vi "RGB to Colour.vi"(8 "error in (no error)":errorcluster, 9 "Blue":u8, 10 "Green":u8, 11 "Red":u8) -> (0 "error out":errorcluster, 3 "Color":u32(colorbox))   [LabVIEW 2018, in "Colour Lab.lvlib"]
uses:
  Colour Lab.lvlib
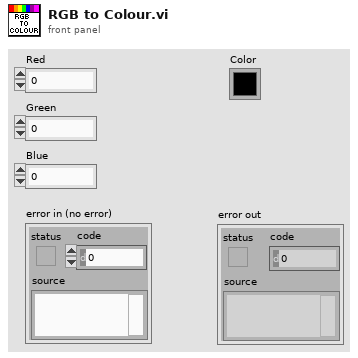
[diagram p1: front panel]
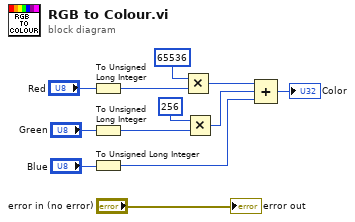
[diagram p0: block diagram]
diagram:
  n1 = To Unsigned Long Integer(number="Red") -> (unsigned 32bit integer=w8:u32)
  n2 = To Unsigned Long Integer(number="Green") -> (unsigned 32bit integer=w6:u32)
  n3 = To Unsigned Long Integer(number="Blue") -> (unsigned 32bit integer=w4:u32)
  n4 = Multiply(x=u32 65536 ("x^2"), y=w8) -> (x*y=w7:u32)
  n5 = Multiply(x=u32 256, y=w6) -> (x*y=w5:u32)
  n6 = Compound Arithmetic op=ADD(w7, w5, w4) -> (→"Color":u32)
  "error out" <- "error in (no error)"
